vi "Add Child.vi"(8 "error in (no error)":errorcluster, 10 "Child":refnum<data-value>, 11 "NodeRef In":refnum<data-value>) -> (0 "error out":errorcluster, 3 "NodeRef":refnum<data-value>)   [LabVIEW 2020, in "PicoG-ParserLexer.lvlib" / "Node.lvclass"]
doc: "Adds the <b>Child</b> node as the first child in the child list of the current node.\n\n<b>Error Codes:</b>\n<b>1556</b>: Nodes must be instantiated with Ctor first."
uses:
  Node.lvclass
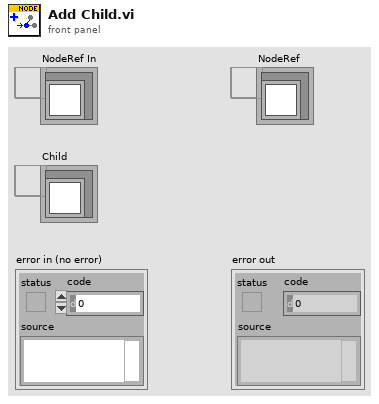
[diagram p1: front panel]
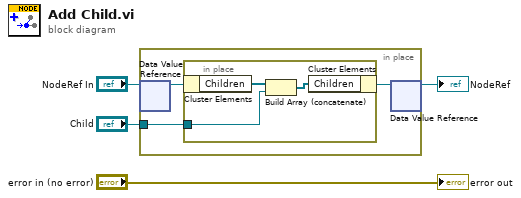
[diagram p0: block diagram]
diagram:
  n1 = in-place {
    in-place-border: "Child" -> [w6]
    n2 = in-place-dvr #1("NodeRef In") -> (w7:refnum<class "Node.lvclass">)  [unwired: 1 out]
    n3 = in-place {
      in-place-border: w6 -> [w9]
      n4 = in-place-cluster #2(w7) -> ("Children"=w10:refnum<data-value>[])
      n5 = Build Array (concatenate)(w10, w9) -> (w8:refnum<data-value>[])
      n6 = in-place-cluster #2("Children"=w8) -> (w5:refnum<class "Node.lvclass">)
    }
    n7 = in-place-dvr #1(w5) -> (→"NodeRef":refnum<data-value>)  [unwired: 1 out]
  }
  "error out" <- "error in (no error)"
